vi "Anal txt open_MS.vi"(7 "Table Tag C":T2, 8 "error in":errorcluster caption="エラー入力", 11 "Table tmp cluster":T1) -> (0 "error out":errorcluster caption="エラー出力", 3 "Table Pass refnum":T3)   [LabVIEW 2018]
panel:
  out "R Table refnum出力":refnum<file>
  out "B Table refnum出力":refnum<file>
  out "S Table refnum出力":refnum<file>
  out "B Table Pass":path
  out "R Table Pass":path
  out "S Table Pass":path
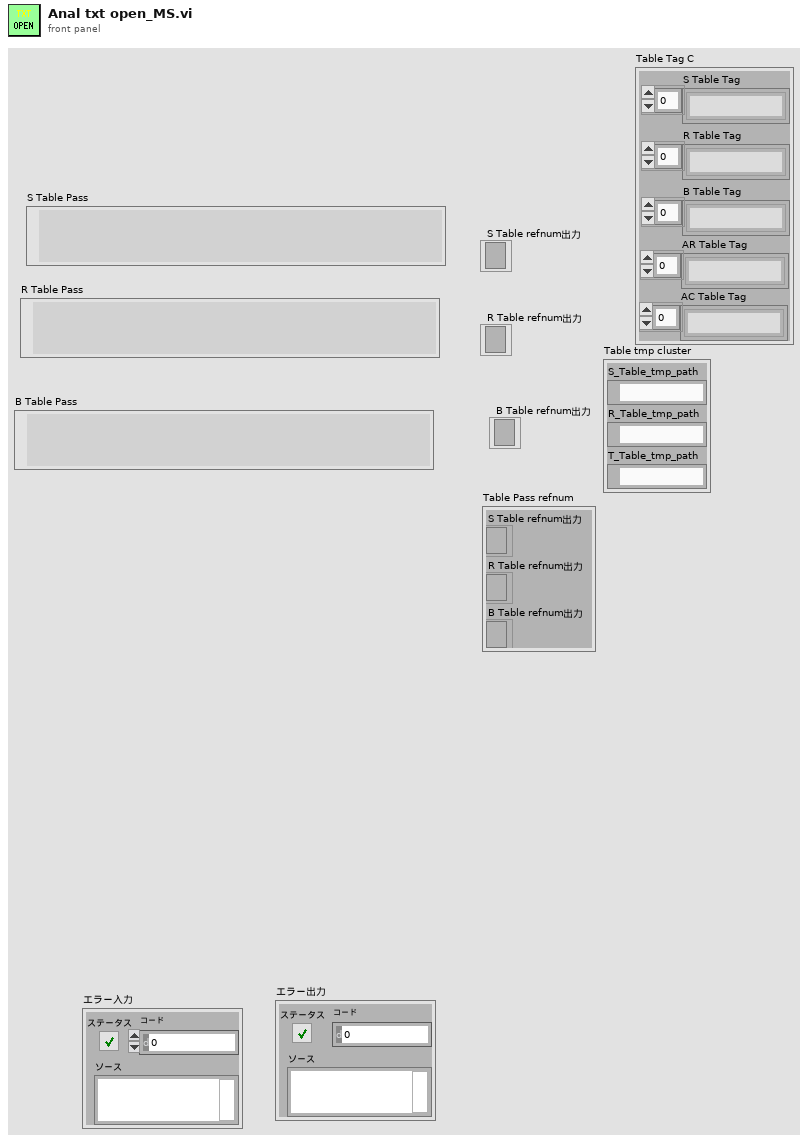
[diagram p1: front panel]
types:
  T1 = cluster{"S_Table_tmp_path":path, "R_Table_tmp_path":path, "T_Table_tmp_path":path}
  T2 = cluster{"S Table Tag":string[], "R Table Tag":string[], "B Table Tag":string[], "AR Table Tag":string[], "AC Table Tag":string[]}
  T3 = cluster{"S Table refnum出力":refnum<file>, "R Table refnum出力":refnum<file>, "B Table refnum出力":refnum<file>}
  T4 = enum16{"open", "replace", "create", "open or create", "replace or create", "replace or create with confirmation"}
  T5 = cluster{"refnum out":refnum<file>, "refnum out":refnum<file>, "refnum out":refnum<file>}
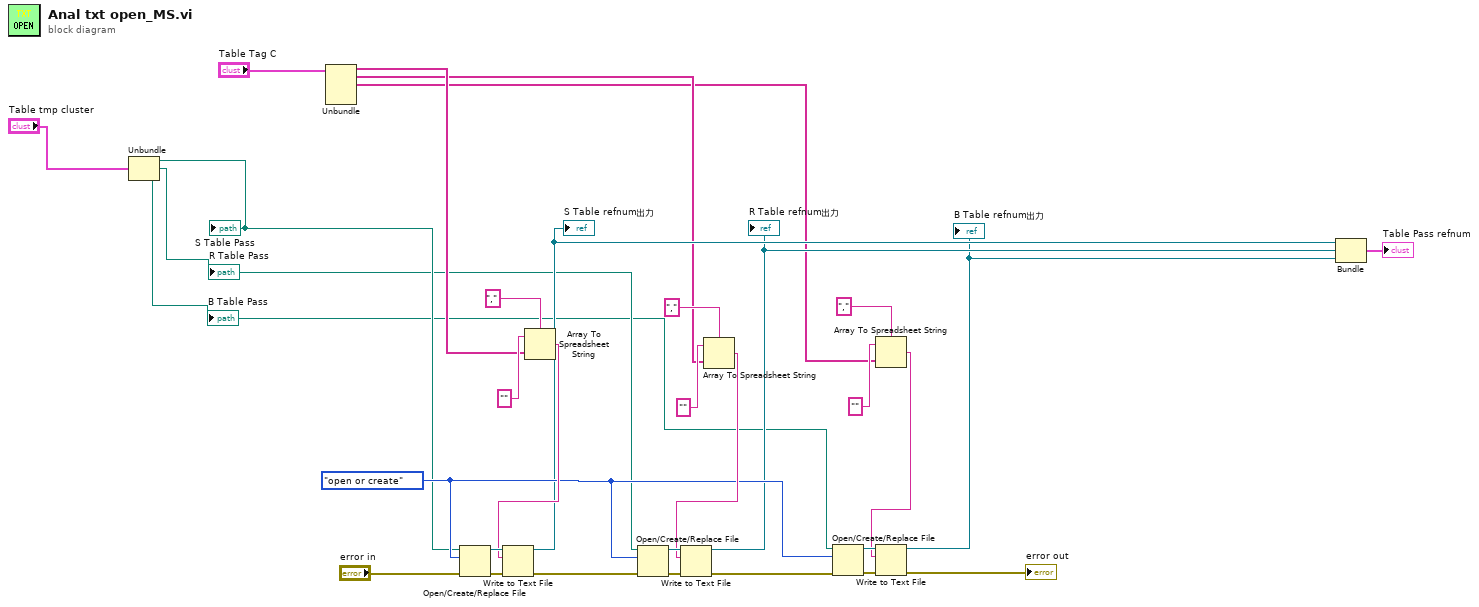
[diagram p0: block diagram]
diagram:
  w19 = T4."open or create" ("操作（0:open）")
  n1 = Unbundle("Table tmp cluster") -> ("S_Table_tmp_path"=w3:path, "R_Table_tmp_path"=w2:path, "T_Table_tmp_path"=w1:path)
  "S Table Pass" <- w3
  "R Table Pass" <- w2
  "B Table Pass" <- w1
  n2 = Unbundle("Table Tag C") -> ("S Table Tag"=w7:string[], "R Table Tag"=w6:string[], "B Table Tag"=w5:string[])  [unwired: 2 out]
  n3 = Open/Create/Replace File(file path (use dialog)=w3, error in="error in", operation (0:open)=w19) -> (refnum out=w29:refnum<file>, error out=w30:errorcluster)  [unwired: 3 in, 1 out]
  n4 = Array To Spreadsheet String(delimiter (Tab)="," ("デリミタ（タブ）"), array=w7, 3:"" ("形式文字列")) -> (spreadsheet string=w27:string)
  n5 = Write to Text File(file (use dialog)=w29, text=w27, error in=w30) -> (refnum out=w11:refnum<file>, error out=w15:errorcluster)  [unwired: 1 in, 1 out]
  "S Table refnum出力" <- w11
  n6 = Open/Create/Replace File(file path (use dialog)=w2, error in=w15, operation (0:open)=w19) -> (refnum out=w25:refnum<file>, error out=w26:errorcluster)  [unwired: 3 in, 1 out]
  n7 = Array To Spreadsheet String(delimiter (Tab)="," ("デリミタ（タブ）"), array=w6, 3:"" ("形式文字列")) -> (spreadsheet string=w20:string)
  n8 = Write to Text File(file (use dialog)=w25, text=w20, error in=w26) -> (refnum out=w10:refnum<file>, error out=w13:errorcluster)  [unwired: 1 in, 1 out]
  "R Table refnum出力" <- w10
  n9 = Open/Create/Replace File(file path (use dialog)=w1, error in=w13, operation (0:open)=w19) -> (refnum out=w23:refnum<file>, error out=w24:errorcluster)  [unwired: 3 in, 1 out]
  n10 = Array To Spreadsheet String(delimiter (Tab)="," ("デリミタ（タブ）"), array=w5, 3:"" ("形式文字列")) -> (spreadsheet string=w16:string)
  n11 = Write to Text File(file (use dialog)=w23, text=w16, error in=w24) -> (refnum out=w9:refnum<file>, error out=→"error out":errorcluster)  [unwired: 1 in, 1 out]
  "B Table refnum出力" <- w9
  n12 = Bundle("refnum out"=w11, "refnum out"=w10, "refnum out"=w9) -> (→"Table Pass refnum":T5)  [unwired: 1 in]
